vi "Call Function with Arrays.vi"(8 "error in (no error)":errorcluster) -> (0 "error out":errorcluster)   [LabVIEW 2020]
uses:
  908d8fb0-7b42-46e8-9e96-a0c6d44c2c93.vi
  G-Embedded-Python-Interpreter-Toolkit/Null Py Object Refnum.vi
  908d8fb0-7b42-46e8-9e96-a0c6d44c2c93.vi/96ddca92-7bbf-40e2-a1a5-d32f291eb6af.vi
  G-Embedded-Python-Interpreter-Toolkit/Python Object Reference to Pointer Sized Ref.vi
  G-Embedded-Python-Interpreter-Toolkit/Pointer Sized Ref to Python Object Reference.vi
  G-Embedded-Python-Interpreter-Toolkit/Generate Function Call Argument Info.vi
  G-Embedded-Python-Interpreter-Toolkit/Bad Type Error.vi
  G-Embedded-Python-Interpreter-Toolkit/Generate Function Call Argument Info.vi/5ba79b4d-2978-48e4-80f3-d9d30d92ebfd.vi
  G-Embedded-Python-Interpreter-Toolkit/Merge Call Library Errors.vi
  <vilib>/Utility/Data Type/Get Type Information.vi
  <vilib>/Utility/error.llb/Error Cluster From Error Code.vi
  <vilib>/Utility/Data Type/Get Cluster Information.vi
  <vilib>/Utility/Data Type/Get Array Information.vi
  <vilib>/addons/_JKI Toolkits/Caraya/classes/Assert/Assert Not Error.vi
  <vilib>/addons/_JKI Toolkits/Caraya/classes/Assert/Assert Equal Value and Type_Variant.vi
  <vilib>/Comparison/Equal/Equal Functor/Equal Functor.lvclass
  G-Embedded-Python-Interpreter-Toolkit/G-Embedded-Python-Interpreter-Toolkit.lvlib
  <vilib>/addons/_JKI Toolkits/Caraya/classes/Test/Test.lvclass
  <vilib>/addons/_JKI Toolkits/Caraya/classes/Assert/Assert.lvclass
panel:
  out "Print Ouptut":string
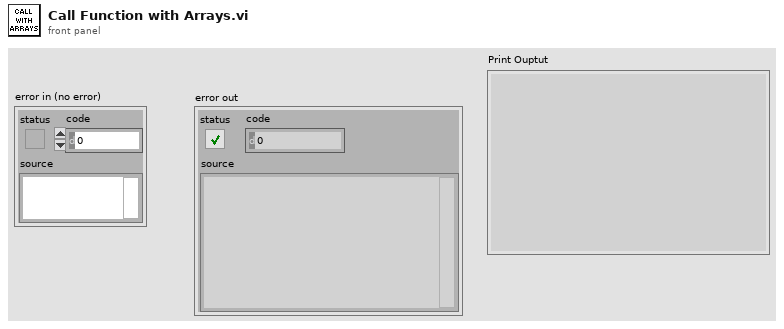
[diagram p1: front panel]
types:
  T1 = typedef "G-Embedded-Python-Interpreter-Toolkit.lvlib/Python Object Reference.ctl" = refnum<k1>
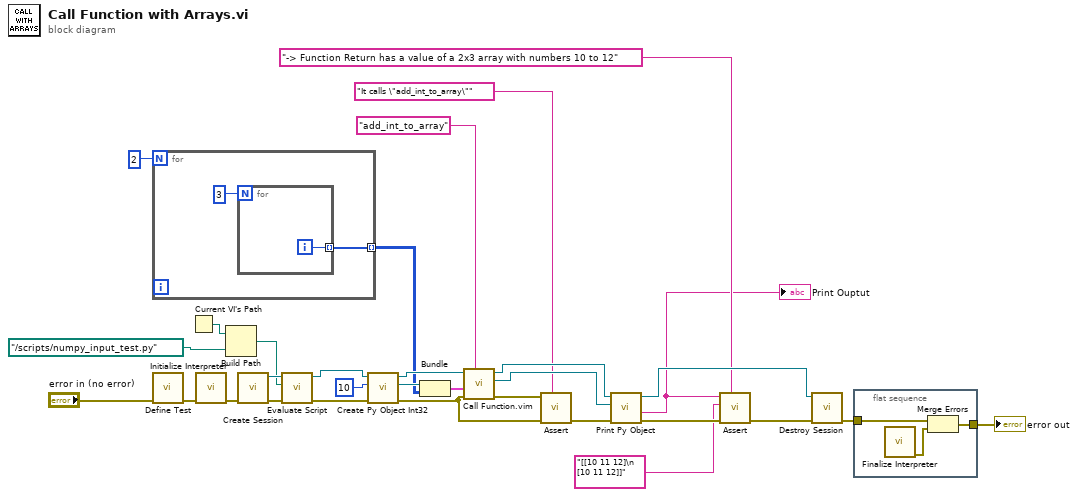
[diagram p0: block diagram]
diagram:
  n1 = for {
    N: 2 -> [_]
    tunnel: [w32] -> w4 mode=indexing
    n2 = for {
      N: 3 -> [_]
      tunnel: [w34] -> w32 mode=indexing
      i -> [w34]
    }
  }
  n3 = call <vilib>:"Define Test.vi"("error in (no error)"="error in (no error)") -> ("error out"=w31:errorcluster)  [unwired: 10 in]
  n4 = Current VI's Path() -> (path=w26:path)
  n5 = call "Initialize Interpreter.vi"("error in (no error)"=w31) -> ("error out"=w28:errorcluster)  [unwired: 9 in, 1 out]
  n6 = Build Path(base path=w26, name or relative path=path "../scripts/numpy_input_test.py" ("Path")) -> (appended path=w24:path)
  n7 = call "Create Session.vi"("error in (no error)"=w28) -> ("error out"=w23:errorcluster, "Session Handle"=w27:refnum<data-value>)  [unwired: 9 in]
  n8 = call "Evaluate Script.vi"("error in (no error)"=w23, "Script File Path"=w24, "Session Handle in"=w27) -> ("error out"=w20:errorcluster, "Session Handle out"=w21:refnum<data-value>)  [unwired: 7 in]
  n9 = call "Create Py Object Int32.vi"("error in (no error)"=w20, "Value"=10, "Session Handle in"=w21) -> ("error out"=w12:errorcluster, "Python Object Refnum"=w5:T1, "Session Handle out"=w19:refnum<data-value>)  [unwired: 6 in]
  n10 = Bundle("Python Object Refnum"=w5, w4) -> (w3:cluster{"Python Object Refnum":T1, i32[][]})  [unwired: 1 in]
  n11 = call "Call Function.vim"("Function Name"="add_int_to_array", "error in (no error)"=w12, "Arguments in (Default - None)"=w3, "Data Value Reference in"=w19) -> ("error out"=w11:errorcluster, "Returned Python Object Refnum"=w17:T1, "Data Value Reference out"=w18:refnum<data-value>)  [unwired: 5 in]
  n12 = call-poly <vilib>:"Assert.vi"("Label"="It calls \"add_int_to_array\"", "error in (no error)"=w12, "Not Error?"=w11) -> ("error out"=w10:errorcluster)  [unwired: 8 in]
  n13 = call "Print Py Object.vi"("error in (no error)"=w10, "Python Object Refnum in"=w17, "Session Handle in"=w18) -> ("error out"=w9:errorcluster, "Print Ouptut"=w2:string, "Session Handle out"=w16:refnum<data-value>)  [unwired: 5 in, 1 out]
  "Print Ouptut" <- w2
  n14 = call-poly <vilib>:"Assert.vi"("Label"="-> Function Return has a value of a 2x3 array with numbers 10 to 12", "error in (no error)"=w9, "Y"="[[10 11 12]\n [10 11 12]]" ("Print Ouptut"), "X"=w2) -> ("error out"=w15:errorcluster)  [unwired: 7 in]
  n15 = call "Destroy Session.vi"("error in (no error)"=w15, "Session Handle"=w16) -> ("error out"=w22:errorcluster)  [unwired: 9 in]
  n16 = flat-sequence {
    tunnel: w22 -> [w37]
    tunnel: [w35] -> w29
    frame #0 {
      n17 = call "Finalize Interpreter.vi"() -> ("error out"=w36:errorcluster)  [unwired: 11 in]
      n18 = Merge Errors(w37, w36) -> (w35:errorcluster)
    }
  }
  "error out" <- w29
